vi "UI-TopWinBlink.vi"(8 "错误输入":errorcluster, 9 "一直置顶？（F）":bool, 10 "闪烁获取焦点(T)":bool=TRUE, 11 "vi ref（TopVIs）":refnum<vi>) -> (0 "错误输出":errorcluster)   [LabVIEW 2017]
doc: "<B>#yyll</B>\n所选VI（不填 Top VI ）窗口闪烁获取焦点，及是否置顶？"
uses:
  user32.dll
panel:
  # "<B>#yyll</B>\n所选VI（不填 Top VI ）窗口闪烁获取焦点，及是否置顶？"
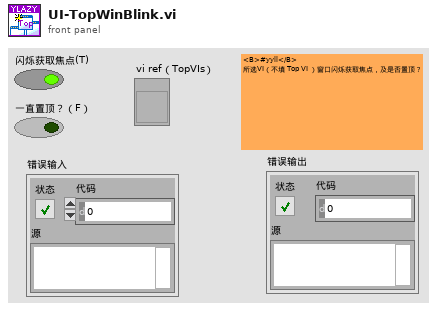
[diagram p1: front panel]
types:
  T1 = enum32{"Invalid", "Standard", "Closed", "Hidden", "Minimized", "Maximized"}
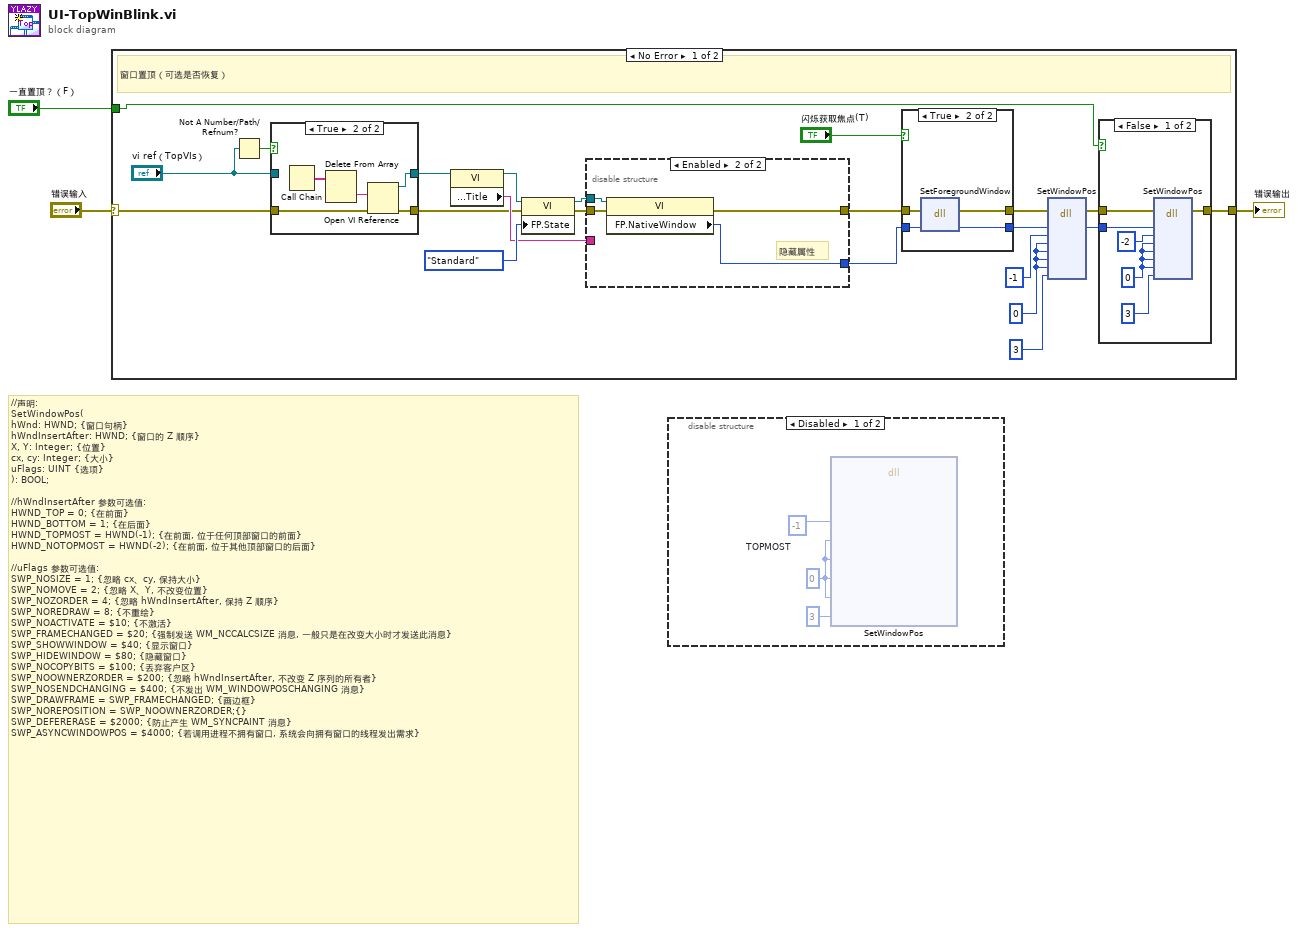
[diagram p0: block diagram]
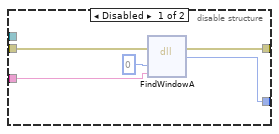
[diagram p4: hidden frame]
diagram:
  # "//声明:\nSetWindowPos(\nhWnd: HWND; {窗口句柄}\nhWndInsertAfter: HWND; {窗口的 Z 顺序}\nX, Y: Integer; {位置}\ncx, cy: Integer; {大小}\nuFlags: UINT {选项}\n): BOOL;\n\n//hWndInsertAfter 参数可选值:\nHWND_TOP = 0; {在前面}\nHWND_BOTTOM = 1; {在后面}\nHWND_TOPMOST = HWND(-1); {在前面, 位于任何顶部窗口的前面}\nHWND_NOTOPMOST = HWND(-2); {在前面, 位于其他顶部窗口的后面}\n\n//uFlags 参数可选值:\nSWP_NOSIZE = 1; {忽略 cx、cy, 保持大小}\nSWP_NOMOVE = 2; {忽略 X、Y, 不改变位置}\nSWP_NOZORDER = 4; {忽略 hWndInsertAfter, 保持 Z 顺序}\nSWP_NOREDRAW = 8; {不重绘}\nSWP_NOACTIVATE = $10; {不激活}\nSWP_FRAMECHANGED = $20; {强制发送 WM_NCCALCSIZE 消息, 一般只是在改变大小时才发送此消息}\nSWP_SHOWWINDOW = $40; {显示窗口}\nSWP_HIDEWINDOW = $80; {隐藏窗口}\nSWP_NOCOPYBITS = $100; {丢弃客户区}\nSWP_NOOWNERZORDER = $200; {忽略 hWndInsertAfter, 不改变 Z 序列的所有者}\nSWP_NOSENDCHANGING = $400; {不发出 WM_WINDOWPOSCHANGING 消息}\nSWP_DRAWFRAME = SWP_FRAMECHANGED; {画边框}\nSWP_NOREPOSITION = SWP_NOOWNERZORDER;{}\nSWP_DEFERERASE = $2000; {防止产生 WM_SYNCPAINT 消息}\nSWP_ASYNCWINDOWPOS = $4000; {若调用进程不拥有窗口, 系统会向拥有窗口的线程发出需求}"
  n1 = case shown="No Error" "错误输入" {
    selector: "错误输入" -> [w25 w55]
    tunnel: [w23 w55] -> w2
    tunnel: "一直置顶？（F）" -> [w15 _]
    frame No Error {
      w20 = 0 ("参数3")
      # "窗口置顶（可选是否恢复）"
      n2 = Not A Number/Path/Refnum?(number/path/refnum="vi ref（TopVIs）") -> (NaN/Path/Refnum?=w5:bool)
      n3 = case shown="True" w5 {
        tunnel: w25 -> [w26 w30]
        tunnel: [w27 w29] -> w14
        tunnel: [w26 w28] -> w11
        tunnel: "vi ref（TopVIs）" -> [w27 _]
        frame False {
        }
        frame True {
          n4 = Call Chain() -> (call chain=w31:string[])
          n5 = Delete From Array(array=w31) -> (deleted portion=w32:string)  [unwired: 2 in, 1 out]
          n6 = Open VI Reference(vi path=w32, error in (no error)=w30) -> (vi reference=w29:refnum<vi>, error out=w28:errorcluster)  [unwired: 4 in]
        }
      }
      n7 = property class="VI"(reference=w14) -> (reference out=w7:refnum<vi>, "Front Panel.Title"=w13:string)  [unwired: 1 in, 1 out]
      n8 = property class="VI"(reference=w7, error in=w11, "FP.State"=T1."Standard" ("Front Panel Window:State")) -> (reference out=w6:refnum<vi>, error out=w9:errorcluster)
      n9 = disable-structure shown="Enabled" {
        disable-tunnel: w13 -> [w36 _]
        disable-tunnel: [w35 w39] -> w12
        disable-tunnel: w9 -> [w34 w40]
        disable-tunnel: [w33 w38] -> w8
        disable-tunnel: w6 -> [_ w41]
        frame Disabled {
          n10 = dll-call lib="user32.dll" fn="FindWindowA" label="FindWindow"(error in=w34, "lpszClassName"=0, "lpszWindowName"=w36) -> (error out=w33:errorcluster, "hWnd"=w35:u32)  [unwired: 4 in, 1 out]
        }
        frame Enabled {
          # "隐藏属性"
          n11 = property class="VI"(reference=w41, error in=w40) -> (error out=w38:errorcluster, "FP.NativeWindow"=w39:u64)  [unwired: 1 out]
        }
      }
      n12 = case shown="True" "闪烁获取焦点(T)" {
        tunnel: [w42 w47] -> w19
        tunnel: w8 -> [w43 w46]
        tunnel: [w43 w45] -> w17
        tunnel: w12 -> [w42 w44]
        frame False {
        }
        frame True {
          n13 = dll-call lib="USER32.DLL" fn="SetForegroundWindow" label="闪烁获取焦点"(error in=w46, "参数1"=w44) -> (error out=w45:errorcluster, "参数1"=w47:u32)  [unwired: 3 in, 1 out]
        }
      }
      n14 = dll-call lib="USER32.DLL" fn="SetWindowPos" label="置顶"(error in=w17, "参数1"=w19, "参数2"=-1, "参数3"=w20, "参数4"=w20, "参数5"=w20, "参数6"=w20, "参数7"=3) -> (error out=w16:errorcluster, "参数1"=w24:u32)  [unwired: 9 in, 1 out]
      n15 = case shown="False" w15 {
        tunnel: w24 -> [w49 _]
        tunnel: [w53 w54] -> w23
        tunnel: w16 -> [w50 w54]
        frame False {
          w52 = 0 ("参数3")
          n16 = dll-call lib="USER32.DLL" fn="SetWindowPos" label="恢复"(error in=w50, "参数1"=w49, "参数2"=-2, "参数3"=w52, "参数4"=w52, "参数5"=w52, "参数6"=w52, "参数7"=3 ("参数3")) -> (error out=w53:errorcluster)  [unwired: 10 in, 1 out]
        }
        frame True {
        }
      }
    }
    frame Error {
    }
  }
  "错误输出" <- w2
  n17 = disable-structure shown="Disabled" {
    frame Disabled {
      w57 = 0 ("参数3")
      w59 = -1  # TOPMOST
      n18 = dll-call lib="USER32.DLL" fn="SetWindowPos" label="置顶"("hWndInsertAfter"=w59, "X"=w57, "Y"=w57, "窗口的新宽度"=w57, "窗口的新高度"=w57, "uFlags"=3 ("参数7")) -> ("hWnd"=w56:u32)  [unwired: 11 in, 2 out]
    }
    frame Enabled {
    }
  }
